vi "Becker-Hickl Decompress LZ4 Data.vi"(8 "Error In":errorcluster, 10 "Uncompressed Block Length":u32, 11 "Compressed Data":u16[](array[numeric]) format="%.0x") -> (0 "Error Out":errorcluster, 3 "Decompressed Data(U16)":u16[](array[numeric]))   [LabVIEW 2021, in "Becker-Hickl Files.lvlib"]
doc: "VI from B&H's software distribution, used to uncompress data compressed with the LZ4 algorithm.\nThis uses two interdependent DLL (the wrapper DLL called in this VI and a LZ4 library saved in the same directory)."
uses:
  Becker-Hickl Files.lvlib
  lz4-wrapper.dll
  <userlib>/_OpenG.lib/array/array.llb/openg_array.lvlib
  <userlib>/_OpenG.lib/array/array.llb/Filter 1D Array (U16)__ogtk.vi
panel:
  out "filtered array":u16[](array[numeric])
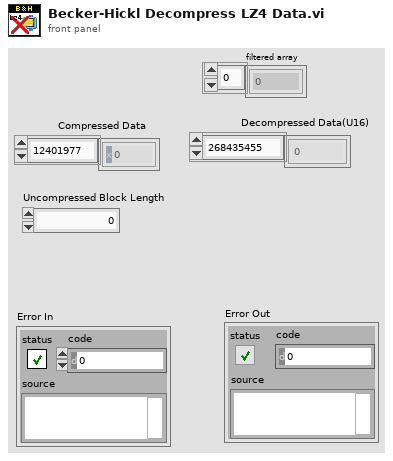
[diagram p1: front panel]
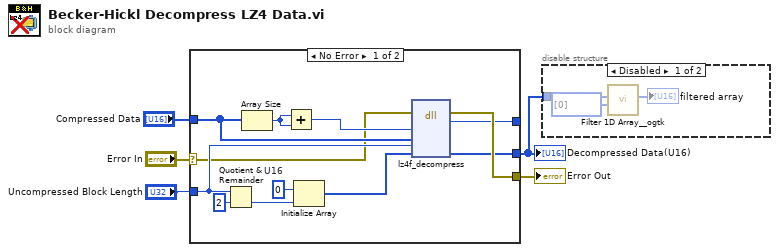
[diagram p0: block diagram]
diagram:
  n1 = case shown="No Error" "Error In" {
    selector: "Error In" -> [w7 w18]
    tunnel: [w14 _] -> w1
    tunnel: [w15 w18] -> w4
    tunnel: "Compressed Data" -> [w8 _]
    tunnel: "Uncompressed Block Length" -> [w11 _]
    tunnel: [w6 _] -> _
    frame No Error {
      w17 = u16 0  # U16
      n2 = Quotient & Remainder(x=w11, y=u32 2) -> (floor(x/y)=w13:u32)  [unwired: 1 out]
      n3 = Array Size(array=w8) -> (size(s)=w9:i32)
      n4 = Add(x=w9, y=w9) -> (x+y=w10:i32)
      n5 = Initialize Array(w17, w13) -> (w16:u16[])
      n6 = dll-call lib="D:/UCLA Thinkpad Google Drive/LabVIEW 2021 SP1/Becker-Hickl Files/lz4-wrapper.dll" fn="lz4f_decompress"(error in=w7, "source_length"=w10, "source_buffer"=w8, "target_length"=w11, "target_buffer"=w16) -> (error out=w15:errorcluster, "return type"=w6:i32, "target_buffer"=w14:u16[])  [unwired: 5 in, 1 out]
    }
    frame Error {
    }
  }
  "Decompressed Data(U16)" <- w1
  "Error Out" <- w4
  n7 = disable-structure shown="Disabled" {
    disable-tunnel: w1 -> [w21 _]
    frame Disabled {
      n8 = call-poly <userlib>:"Filter 1D Array__ogtk.vi"("items to filter"=u16[] [0], "array"=w21) -> ("filtered array"=→"filtered array":u16[])  [unwired: 4 in, 1 out]
    }
    frame Enabled {
    }
  }
